vi "VIH HelpGen - Get PolyVI Instance VI Paths.vi"(8 "error in":errorcluster, 10 "VI Path":path, 11 "VI Reference":refnum<vi>) -> (0 "error out":errorcluster, 2 "Instance VI Paths":path[](array[path]), 3 "dup VI Reference":refnum<vi>)   [LabVIEW 2014]
doc: "::: VI Helpeks :::\nCopyright (c) 2000-2026 Konstantin Shifershteyn. All rights reserved."
panel:
  # "VI Helpeks\nCopyright (c) 2012-2026 Konstantin Shifershteyn"
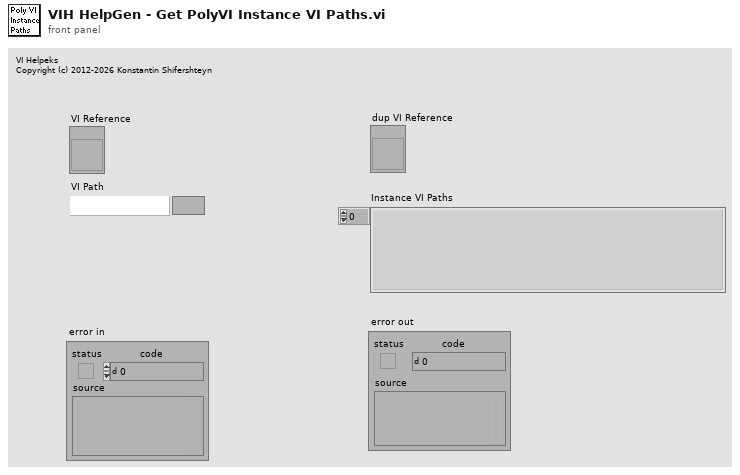
[diagram p1: front panel]
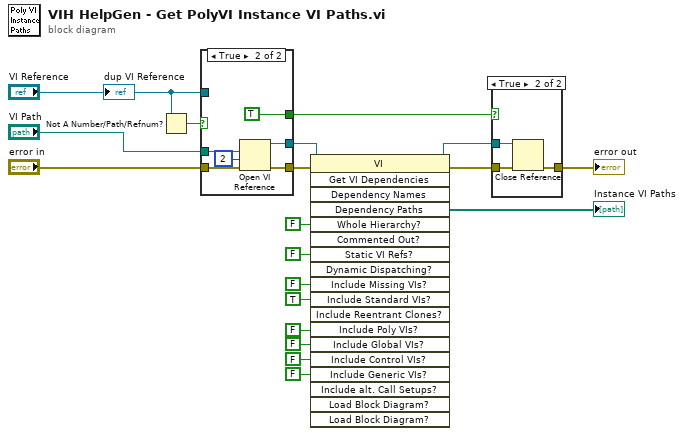
[diagram p0: block diagram]
diagram:
  n1 = Not A Number/Path/Refnum?(number/path/refnum="VI Reference") -> (NaN/Path/Refnum?=w8:bool)
  n2 = case shown="True" w8 {
    tunnel: [w20 w27] -> w11
    tunnel: [w21 w26] -> w10
    tunnel: "VI Path" -> [_ w25]
    tunnel: "VI Reference" -> [w21 _]
    tunnel: "error in" -> [w20 w24]
    tunnel: [_ TRUE] -> w3
    frame False {
    }
    frame True {
      n3 = Open VI Reference(vi path=w25, options=2, error in (no error)=w24) -> (vi reference=w26:refnum<vi>, error out=w27:errorcluster)  [unwired: 3 in]
    }
  }
  n4 = invoke class="VI" method="Get VI Dependencies"(reference=w10, error in=w11, "Whole Hierarchy?"=FALSE, "Static VI Refs?"=FALSE, "Include Missing VIs?"=FALSE ("Include Missing Items?"), "Include Standard VIs?"=TRUE, "Include Poly VIs?"=FALSE, "Include Global VIs?"=FALSE, "Include Control VIs?"=FALSE, "Include Generic VIs?"=FALSE) -> (reference out=w1:refnum<vi>, error out=w5:errorcluster, "Dependency Paths"=→"Instance VI Paths":path[])  [unwired: 9 in, 16 out]
  n5 = case shown="True" w3 {
    tunnel: w5 -> [w28 w31]
    tunnel: [w28 w30] -> w4
    tunnel: w1 -> [_ w29]
    frame False {
    }
    frame True {
      n6 = Close Reference(reference=w29, error in (no error)=w31) -> (error out=w30:errorcluster)
    }
  }
  "error out" <- w4
  "dup VI Reference" <- "VI Reference"
